vi "[ce low] Find Local Zero, Min or Max.vi"(4 "find":enum16{"zero", "min", "max"}(ring), 5 "# points":u32=100, 6 "accuracy":dbl=1e-08 format="%.2e", 7 "VC Handle":T1=-1, 8 "error in":errorcluster, 9 "formula info":cluster{"formula":string, "x-variable":string}={"formula"="", "x-variable"="t"}, 10 "end":dbl=1.0 format="%.6e", 11 "start":dbl format="%.6e") -> (0 "error out":errorcluster, 2 "f(x)":dbl format="%.9e", 3 "x":dbl format="%.9e")   [LabVIEW 2021]
doc: "::: CalcExpress Toolkit :::\nCopyright (c) 2000-2026 Konstantin Shifershteyn. All rights reserved."
uses:
  cetypes.llb/VarMan Variable Context Handle.ctl
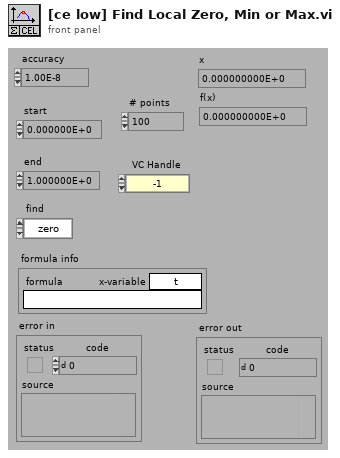
[diagram p1: front panel]
types:
  T1 = typedef "VarMan Variable Context Handle.ctl" = i32
  T2 = enum16{"create", "destroy", "set value", "get value"}
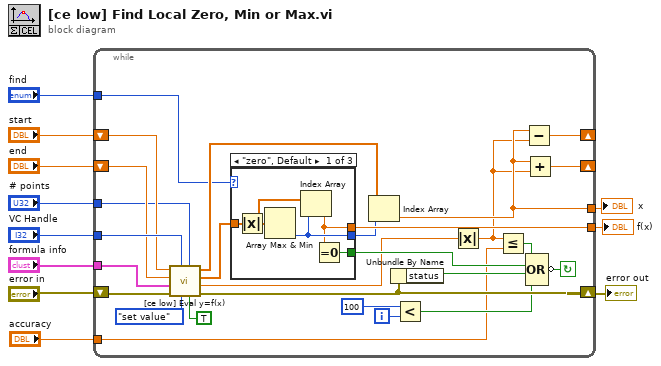
[diagram p0: block diagram]
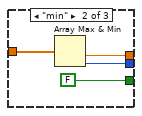
[diagram p2: hidden frame]
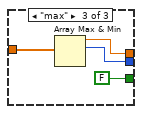
[diagram p3: hidden frame]
diagram:
  n1 = while {
    tunnel: "accuracy" -> [w18]
    tunnel: "VC Handle" -> [w36]
    tunnel: [w24] -> w6
    tunnel: "formula info" -> [w37]
    tunnel: "# points" -> [w15]
    tunnel: [w28] -> w10
    shift-left: "end" -> [w34]
    shift-right: [w26] -> _
    shift-left: "start" -> [w35]
    shift-right: [w27] -> _
    shift-left: "error in" -> [w38]
    shift-right: [w25] -> w9
    tunnel: "find" -> [w12]
    i -> [w32]
    stop <- w33 continue-if-true
    n2 = call "[ce low] Eval y=f(x).vi"("include end point"=TRUE ("extend range"), "# points"=w15, "vm cmd"=T2."set value", "VC Handle"=w36, "error in"=w38, "formula info"=w37, "end"=w34, "start"=w35) -> ("error out"=w25:errorcluster, "dx"=w14:dbl, "f(x)"=w29:dbl[], "x"=w13:dbl[])
    n3 = case shown="\"zero\", Default" w12 {
      tunnel: w29 -> [w43 w47 w51]
      tunnel: [w40 w46 w50] -> w24
      tunnel: [w41 w45 w49] -> w23
      tunnel: [w39 FALSE FALSE] -> w19
      frame "zero", Default {
        n4 = Absolute Value(x=w43) -> (abs(x)=w42:dbl[])
        n5 = Array Max & Min(array=w42) -> (min index (indices)=w41:i32)  [unwired: 3 out]
        n6 = Index Array(array=w43, index=w41) -> (element=w40:dbl)
        n7 = Equal To 0?(x=w40) -> (x = 0?=w39:bool)
      }
      frame "min" {
        n8 = Array Max & Min(array=w47) -> (min value=w46:dbl, min index (indices)=w45:i32)  [unwired: 2 out]
      }
      frame "max" {
        n9 = Array Max & Min(array=w51) -> (max value=w50:dbl, max index (indices)=w49:i32)  [unwired: 2 out]
      }
    }
    n10 = Index Array(array=w13, index=w23) -> (element=w28:dbl)
    n11 = Unbundle By Name(w25) -> ("status"=w21:bool)
    n12 = Less?(x=100, y=w32) -> (x < y?=w20:bool)
    n13 = Absolute Value(x=w14) -> (abs(x)=w22:dbl)
    n14 = Less Or Equal?(x=w22, y=w18) -> (x <= y?=w16:bool)
    n15 = Subtract(x=w28, y=w22) -> (x-y=w27:dbl)
    n16 = Add(x=w28, y=w22) -> (x+y=w26:dbl)
    n17 = Compound Arithmetic op=OR(w16, w19, w21, w20) -> (invert w33:bool)
  }
  "x" <- w10
  "error out" <- w9
  "f(x)" <- w6
